vi "Open Debug Process.vi"(7 "Process":refnum<vi>, 8 "error in (no error)":errorcluster, 9 "Open panel?":bool, 10 "New instance?":bool, 11 "DebuggingTerminal in":refnum<class "DebuggingTerminal.lvclass">) -> (0 "error out":errorcluster, 1 "VI Refnum":refnum<vi>, 3 "DebuggingTerminal out":refnum<class "DebuggingTerminal.lvclass">)   [LabVIEW 2013, in "MQTT Base.lvlib" / "DebuggingTerminal.lvclass"]
uses:
  DebuggingTerminal.lvclass
  DebuggingTerminal.lvclass/DebuggingTerminal.ctl
  MQTT Base.lvlib
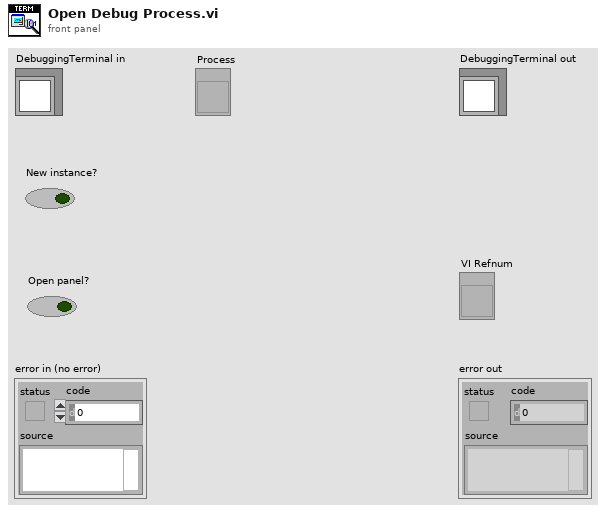
[diagram p1: front panel]
types:
  T1 = enum32{"Bad", "Idle", "Run top level", "Running"}
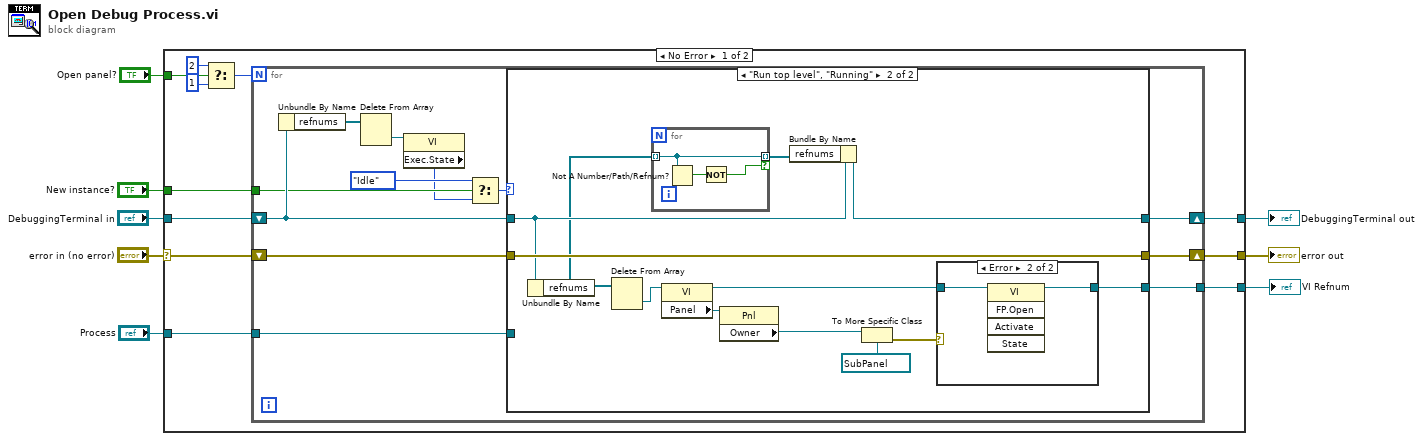
[diagram p0: block diagram]
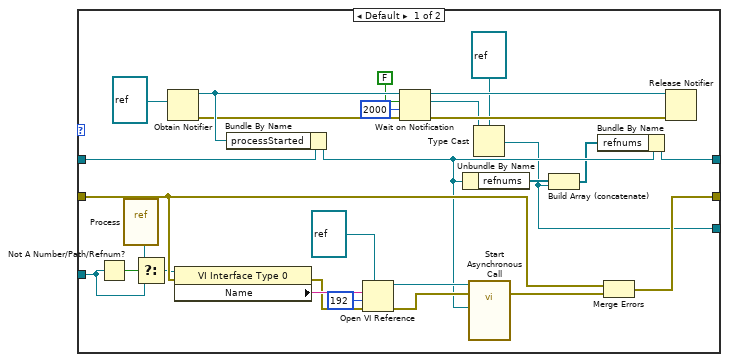
[diagram p2: hidden frame]
diagram:
  n1 = case shown="No Error" "error in (no error)" {
    selector: "error in (no error)" -> [w19 w79]
    tunnel: [w18 w79] -> w7
    tunnel: [w17 w78] -> w5
    tunnel: "DebuggingTerminal in" -> [w16 w78]
    tunnel: "Open panel?" -> [w15 _]
    tunnel: "Process" -> [w11 _]
    tunnel: [w10 _] -> w2
    tunnel: "New instance?" -> [w9 _]
    frame No Error {
      n2 = Select(t=2, s=w15, f=1) -> (s? t:f=w12:i32)
      n3 = for {
        N: w12 -> [_]
        shift-right: [w29] -> w17
        shift-left: w16 -> [w28]
        shift-right: [w30] -> w18
        shift-left: w19 -> [w31]
        tunnel: w11 -> [w27]
        tunnel: [w26] -> w10
        tunnel: w9 -> [w23]
        n4 = Unbundle By Name(w28) -> ("refnums"=w25:refnum<vi>[])
        n5 = Delete From Array(array=w25) -> (deleted portion=w24:refnum<vi>)  [unwired: 2 in, 1 out]
        n6 = property class="VI"(reference=w24) -> ("Exec.State"=w21:T1)  [unwired: 1 in, 2 out]
        n7 = Select(t=T1."Idle", s=w23, f=w21) -> (s? t:f=w20:T1)
        n8 = case shown="\"Run top level\", \"Running\"" w20 {
          tunnel: w31 -> [w54 w71]
          tunnel: [w53 w71] -> w30
          tunnel: [w45 w61] -> w29
          tunnel: w28 -> [w44 w62]
          tunnel: w27 -> [w37 _]
          tunnel: [w32 w70] -> w26
          frame Default {
            n9 = Not A Number/Path/Refnum?(number/path/refnum=w37) -> (NaN/Path/Refnum?=w39:bool)
            n10 = vi-ref "Process.vi"() -> (w38:refnum<vi>)
            n11 = Select(t=w38, s=w39, f=w37) -> (s? t:f=w36:refnum<vi>)
            n12 = Obtain Notifier(notification data type=refnum<vi> refnum ("This VI")) -> (notifier out=w50:refnum<notifier>, error out=w47:errorcluster)  [unwired: 3 in, 1 out]
            n13 = property class="VI Interface Type 0"(reference=w36, error in=w54) -> (error out=w56:errorcluster, "Name"=w57:string)  [unwired: 1 out]
            n14 = Bundle By Name(cluster=w44, "processStarted"=w50) -> (w35:refnum<class "DebuggingTerminal.lvclass">)
            n15 = Open VI Reference(type specifier VI Refnum (for type only)=refnum<vi> refnum, vi path=w57, options=192, error in (no error)=w56) -> (vi reference=w59:refnum<vi>, error out=w51:errorcluster)  [unwired: 2 in]
            n16 = Wait on Notification(notifier=w50, ignore previous (F)=FALSE, timeout in ms (-1)=2000, error in (no error)=w47) -> (notifier out=w48:refnum<notifier>, notification=w42:refnum<vi>, error out=w49:errorcluster)  [unwired: 1 out]
            n17 = Unbundle By Name(w35) -> ("refnums"=w34:refnum<vi>[])
            n18 = call-by-ref "Start Asynchronous Call"(reference=w59, error in=w51, "DebuggingTerminal"=w35) -> (error out=w55:errorcluster)  [unwired: 11 in, 1 out]
            n19 = Type Cast(type=refnum<vi> refnum ("refnum"), x=w42) -> (*(type *) &x=w32:refnum<vi>)
            n20 = Build Array (concatenate)(w34, w32) -> (w33:refnum<vi>[])
            n21 = Bundle By Name(cluster=w35, "refnums"=w33) -> (w45:refnum<class "DebuggingTerminal.lvclass">)
            n22 = Merge Errors(w54, w55) -> (w53:errorcluster)
            n23 = Release Notifier(notifier=w48, error in (no error)=w49) -> ()  [unwired: 1 in, 3 out]
          }
          frame "Run top level", "Running" {
            n24 = Unbundle By Name(w62) -> ("refnums"=w60:refnum<vi>[])
            n25 = Delete From Array(array=w60) -> (deleted portion=w69:refnum<vi>)  [unwired: 2 in, 1 out]
            n26 = for {
              tunnel: w60 -> [w74] mode=indexing
              tunnel: [w74] -> w63 mode=indexing if=w72
              n27 = Not A Number/Path/Refnum?(number/path/refnum=w74) -> (NaN/Path/Refnum?=w73:bool)
              n28 = Not(x=w73) -> (.not. x?=w72:bool)
            }
            n29 = property class="VI"(reference=w69) -> (reference out=w68:refnum<vi>, "Panel"=w67:refnum<vi>)  [unwired: 1 in, 1 out]
            n30 = property class="Pnl"(reference=w67) -> ("Owner"=w66:refnum<vi>)  [unwired: 1 in, 2 out]
            n31 = Bundle By Name(cluster=w62, "refnums"=w63) -> (w61:refnum<class "DebuggingTerminal.lvclass">)
            n32 = To More Specific Class(target class=refnum<vi> refnum ("Owner"), reference=w66) -> (error out=w64:errorcluster)  [unwired: 1 in, 1 out]
            n33 = case shown="Error" w64 {
              tunnel: [w75 w77] -> w70
              tunnel: w68 -> [w75 w76]
              frame No Error {
              }
              frame Error {
                n34 = invoke class="VI" method="FP.Open"(reference=w76) -> (reference out=w77:refnum<vi>)  [unwired: 4 in, 4 out]
              }
            }
          }
        }
      }
    }
    frame Error {
    }
  }
  "error out" <- w7
  "DebuggingTerminal out" <- w5
  "VI Refnum" <- w2
